vi "Format Word for CSV.vi"(10 "data word format":T1="Hexadecimal", 11 "Word":T2) -> (3 "String Array":string[](array[string]))   [LabVIEW 2020, in "Ballard ARINC 429 Engine.lvlib" / "Implementation.lvlib" / "CSV Word Logger.lvclass"]
uses:
  CSV Word Logger.lvclass
  Word.ctl
  Shared/Data Word Format.ctl
  Implementation.lvlib
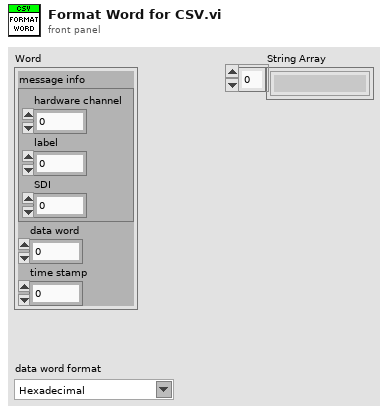
[diagram p1: front panel]
types:
  T1 = typedef "Data Word Format.ctl" = string
  T2 = typedef "Ballard ARINC 429 Engine.lvlib/Implementation.lvlib/Word.ctl" = cluster{"message info":cluster{"hardware channel":u8, "label":u8, "SDI":u8}, "data word":u32, "time stamp":dbl}
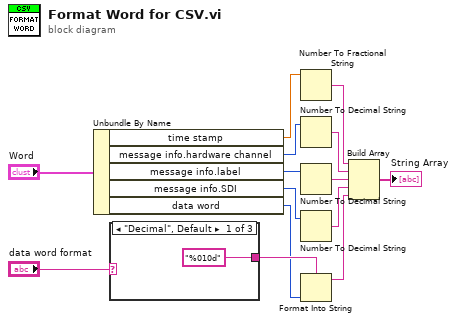
[diagram p0: block diagram]
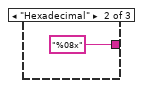
[diagram p2: hidden frame]
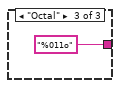
[diagram p3: hidden frame]
diagram:
  n1 = Unbundle By Name("Word") -> ("time stamp"=w6:dbl, "message info.hardware channel"=w5:u8, "message info.label"=w4:u8, "message info.SDI"=w3:u8, "data word"=w12:u32)
  n2 = case shown="\"Decimal\", Default" "data word format" {
    tunnel: ["%010d" ("format string") "%08x" ("format string") "%011o" ("format string")] -> w14
    frame "Decimal", Default {
    }
    frame "Hexadecimal" {
    }
    frame "Octal" {
    }
  }
  n3 = Number To Fractional String(number=w6) -> (F-format string=w10:string)  [unwired: 3 in]
  n4 = Number To Decimal String(number=w5) -> (decimal integer string=w7:string)  [unwired: 1 in]
  n5 = Number To Decimal String(number=w4) -> (decimal integer string=w9:string)  [unwired: 1 in]
  n6 = Number To Decimal String(number=w3) -> (decimal integer string=w8:string)  [unwired: 1 in]
  n7 = Format Into String(format string=w14, w12) -> (resulting string=w13:string)  [unwired: 2 in, 1 out]
  n8 = Build Array(w10, w7, w9, w8, w13) -> (→"String Array":string[])
